vi "Genertate Menu.vi"(8 "error in (no error)":errorcluster caption="错误输入（无错误）", 10 "菜单引用":refnum<k9>, 11 "Data Viewer 输入":refnum<class "Data Viewer.lvclass">) -> (0 "error out":errorcluster caption="错误输出", 3 "Data Viewer 输出":refnum<class "Data Viewer.lvclass">)   [LabVIEW 2020, in "Data Viewer.lvlib" / "Data Viewer.lvclass"]
uses:
  Data Viewer.lvclass
  Data Viewer.lvclass/Data Viewer.ctl
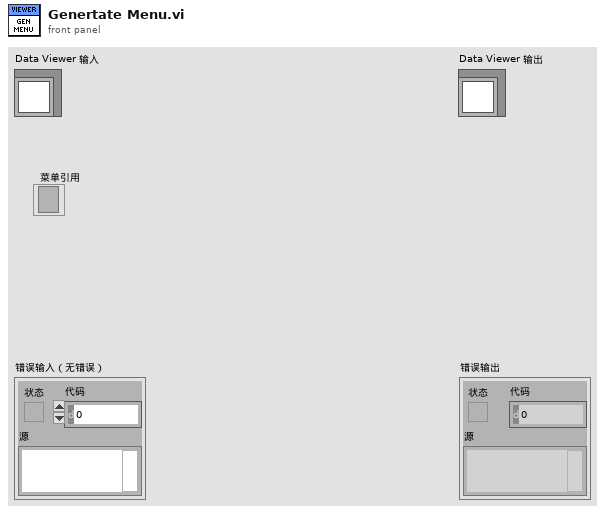
[diagram p1: front panel]
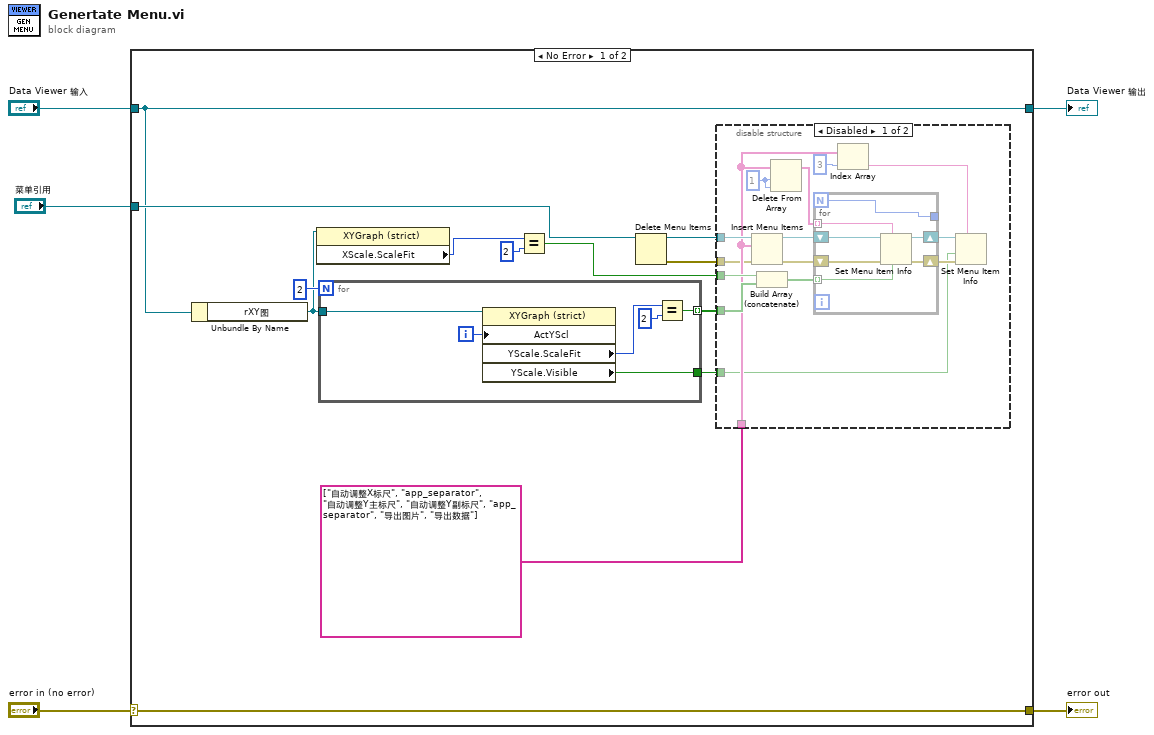
[diagram p0: block diagram]
diagram:
  n1 = case shown="No Error" "error in (no error)" {
    selector: "error in (no error)" -> [w18 w48]
    tunnel: [w18 w48] -> w4
    tunnel: [w15 w47] -> w2
    tunnel: "Data Viewer 输入" -> [w15 w47]
    tunnel: "菜单引用" -> [w17 _]
    frame No Error {
      n2 = Unbundle By Name(w15) -> ("rXY图"=w7:refnum<vi>)
      n3 = property class="XYGraph (strict)"(reference=w7) -> ("XScale.ScaleFit"=w13:u8)  [unwired: 1 in, 2 out]
      n4 = for {
        N: 2 -> [_]
        tunnel: w7 -> [w46]
        tunnel: [w43] -> w10 mode=indexing
        tunnel: [w41] -> w6
        i -> [w42]
        n5 = property class="XYGraph (strict)"(reference=w46, "ActYScl"=w42) -> ("YScale.ScaleFit"=w44:u8, "YScale.Visible"=w41:bool)  [unwired: 1 in, 2 out]
        n6 = Equal?(x=w44, y=u8 2) -> (x = y?=w43:bool)
      }
      n7 = Equal?(x=w13, y=u8 2) -> (x = y?=w11:bool)
      n8 = Delete Menu Items(9:w17) -> (0:w8:errorcluster, 3:w16:refnum<k9>)  [unwired: 3 in]
      n9 = disable-structure shown="Disabled" {
        disable-tunnel: w16 -> [w33 _]
        disable-tunnel: w11 -> [w29 _]
        disable-tunnel: w10 -> [w28 _]
        disable-tunnel: string[] ["自动调整X标尺", "app_separator", "自动调整Y主标尺", "自动调整Y副标尺", "app_separator", "导出图片", "导出数据"] ("项名称") -> [w25 _]
        disable-tunnel: w8 -> [w22 _]
        disable-tunnel: w6 -> [w19 _]
        frame Disabled {
          w31 = 1 ("长度")
          n10 = Insert Menu Items(6:w22, 8:w25, 9:w33) -> (0:w21:errorcluster, 3:w32:refnum<k9>)  [unwired: 3 in, 1 out]
          n11 = Build Array (concatenate)(w29, w28) -> (w27:bool[])
          n12 = Delete From Array(array=w25, length=w31, index=w31) -> (array with subset deleted=w30:string[])  [unwired: 1 out]
          n13 = for {
            N -> [w36]
            tunnel: w30 -> [w38] mode=indexing
            tunnel: w27 -> [w39] mode=indexing
            shift-right: [w37] -> w26
            shift-left: w32 -> [w40]
            tunnel: [w36] -> _
            shift-right: [w34] -> w20
            shift-left: w21 -> [w35]
            n14 = Set Menu Item Info(6:w39, 7:w38, 8:w35, 11:w40) -> (0:w34:errorcluster, 3:w37:refnum<k9>)  [unwired: 3 in]
          }
          n15 = Index Array(array=w25, index=3 ("索引")) -> (element=w23:string)
          n16 = Set Menu Item Info(7:w23, 8:w20, 9:w19, 11:w26) -> ()  [unwired: 3 in, 2 out]
        }
        frame Enabled {
        }
      }
    }
    frame Error {
    }
  }
  "error out" <- w4
  "Data Viewer 输出" <- w2
